vi "SMD trans.vi"(8 "error in (no error) 2":errorcluster, 11 "Disturb":bool) -> (0 "error in (no error) 3":errorcluster, 3 "Acceleration":dbl)   [LabVIEW 2026]
doc: "Ths VI calculates the transient response based on an exponentially decaying sinusoid. When disturb is true it creates an initial acceleration and its derivitive. When Disturb is false, it gives you the current acceleation"
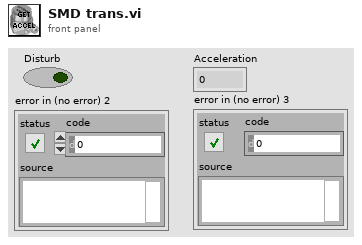
[diagram p1: front panel]
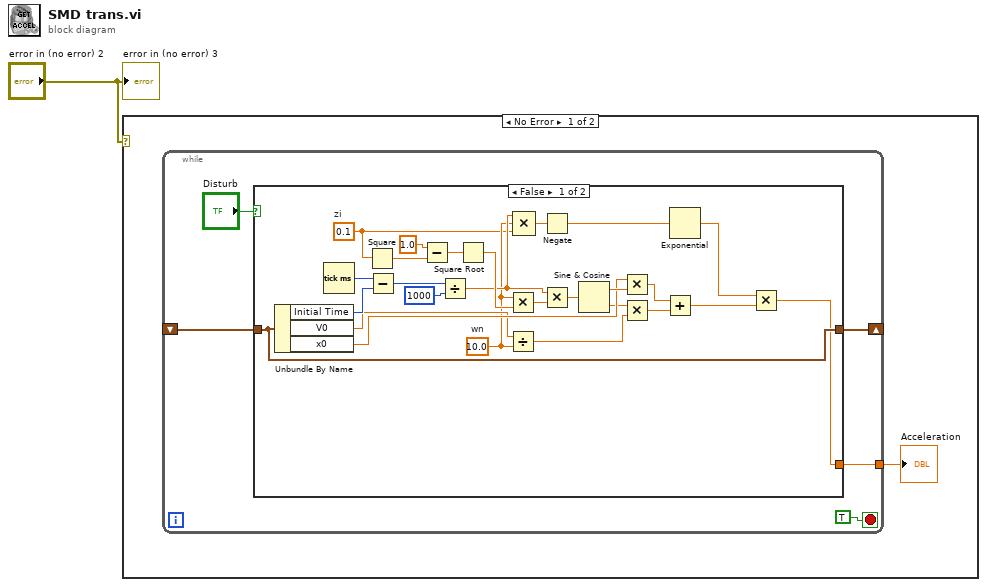
[diagram p0: block diagram]
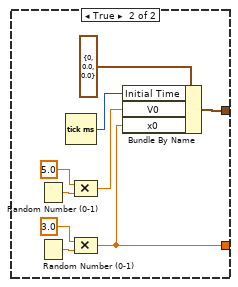
[diagram p2: hidden frame]
diagram:
  n1 = case shown="No Error" "error in (no error) 2" {
    frame No Error {
      n2 = while {
        shift-right: [w7] -> _
        shift-left: _ -> [w4]
        tunnel: [w5] -> w2
        stop <- TRUE stop-if-true
        n3 = case shown="False" "Disturb" {
          tunnel: [w33 w41] -> w7
          tunnel: [w14 w34] -> w5
          tunnel: w4 -> [w33 _]
          frame False {
            w11 = 0.1  # zi
            w12 = 10.0  # wn
            n4 = Unbundle By Name(w33) -> ("Initial Time"=w32:u32, "V0"=w20:dbl, "x0"=w21:dbl)
            n5 = Tick Count (ms)() -> (millisecond timer value=w31:u32)
            n6 = Square(x=w11) -> (x^2=w27:dbl)
            n7 = Subtract(x=w31, y=w32) -> (x-y=w30:u32)
            n8 = Subtract(x=1.0, y=w27) -> (x-y=w26:dbl)
            n9 = Divide(x=w30, y=u32 1000) -> (x/y=w13:dbl)
            n10 = Square Root(x=w26) -> (sqrt(x)=w25:dbl)
            n11 = Multiply(x=w12, y=w25) -> (x*y=w24:dbl)
            n12 = Divide(x=w20, y=w12) -> (x/y=w18:dbl)
            n13 = Compound Arithmetic op=MULTIPLY(w13, w12, w11) -> (w10:dbl)
            n14 = Negate(x=w10) -> (-x=w9:dbl)
            n15 = Multiply(x=w13, y=w24) -> (x*y=w23:dbl)
            n16 = Sine & Cosine(0:w23) -> (1:w22:dbl, 2:w19:dbl)
            n17 = Multiply(x=w21, y=w22) -> (x*y=w17:dbl)
            n18 = Multiply(x=w19, y=w18) -> (x*y=w16:dbl)
            n19 = Add(x=w17, y=w16) -> (x+y=w15:dbl)
            n20 = Exponential(1:w9) -> (0:w8:dbl)
            n21 = Multiply(x=w8, y=w15) -> (x*y=w14:dbl)
          }
          frame True {
            n22 = Random Number (0-1)() -> (number: 0 to 1=w39:dbl)
            n23 = Random Number (0-1)() -> (number: 0 to 1=w35:dbl)
            n24 = Tick Count (ms)() -> (millisecond timer value=w40:u32)
            n25 = Compound Arithmetic op=MULTIPLY(5.0 ("value"), w39) -> (w38:dbl)
            n26 = Compound Arithmetic op=MULTIPLY(3.0 ("value"), w35) -> (w34:dbl)
            n27 = Bundle By Name(cluster=cluster{"Initial Time":u32, "V0":dbl, "x0":dbl} {"Initial Time"=0, "V0"=0.0, "x0"=0.0} ("Cluster"), "Initial Time"=w40, "V0"=w38, "x0"=w34) -> (w41:cluster{"Initial Time":u32, "V0":dbl, "x0":dbl})
          }
        }
      }
      "Acceleration" <- w2
    }
    frame Error {
    }
  }
  "error in (no error) 3" <- "error in (no error) 2"
